vi "run-tests.vi"() -> ()   [LabVIEW 2026]
doc: "Caraya suite runner\\2C generated by lvai_generate_caraya_test_runner.\\0A\\0AIt builds every test VI's path relative to its OWN location\\2C so the suite moves with the folder\\2C and runs them through Caraya's Run Tests.vi (Array Path instance) with Interactive FALSE - a TRUE there opens a modal report dialog\\2C which stops LabVIEW's gRPC service until a human dismisses it.\\0A\\0ARead the JUnit report named by 'Report Path used'\\2C not 'error out'\\3A the error cluster carries the FIRST failed assertion only."
uses:
  <vilib>/addons/_JKI Toolkits/Caraya/Caraya.lvlib
panel:
  out "error out":errorcluster
  out "Report Path used":path
  in  "error in":errorcluster
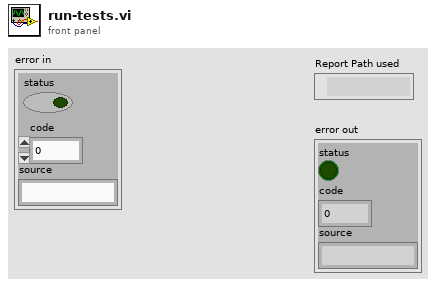
[diagram p1: front panel]
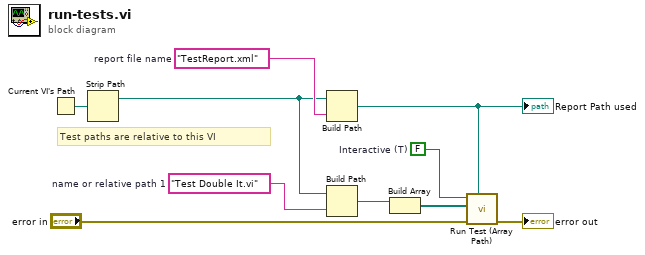
[diagram p0: block diagram]
diagram:
  w8 = FALSE  # Interactive (T)
  w4 = "TestReport.xml"  # report file name
  w3 = "Test Double It.vi"  # name or relative path 1
  # "Test paths are relative to this VI"
  n1 = Current VI's Path() -> (path=w1:path)
  n2 = Strip Path(path=w1) -> (stripped path=w2:path)  [unwired: 1 out]
  n3 = Build Path(base path=w2, name or relative path=w4) -> (appended path=w6:path)
  "Report Path used" <- w6
  n4 = Build Path(base path=w2, name or relative path=w3) -> (appended path=w5:path)
  n5 = Build Array(w5) -> (w7:path[])
  n6 = call <vilib>:"Run Test (Array Path).vi"("Report Path"=w6, "error in"="error in", "Paths"=w7, "Interactive (T)"=w8) -> ("error out"=→"error out":errorcluster)  [unwired: 6 in, 1 out]
